vi "Deposit Funds.vi"(8 "error in":errorcluster, 9 "Amount":dbl, 10 "Account Number":string, 11 "Accounts File Path":path) -> (0 "error out":errorcluster, 3 "Account":T1)   [LabVIEW 2026]
doc: "Deposits Amount into an account. The CURRENT balance is read from the accounts file (Get Account.vi), Amount is added and the new balance is written back with Update Account Balance.vi; Account returns the updated record. An account number that is not in the file returns error 5003 and nothing is written. When error in carries an error the file is neither read nor written."
uses:
  Controls/ATM Account.ctl
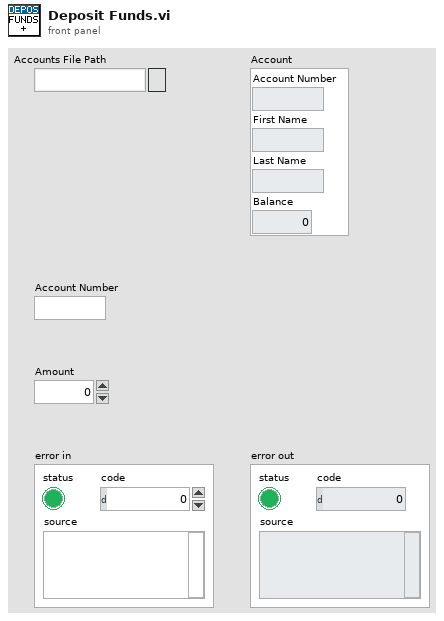
[diagram p1: front panel]
types:
  T1 = typedef "ATM Account.ctl" = cluster{"Account Number":string, "First Name":string, "Last Name":string, "Balance":dbl}
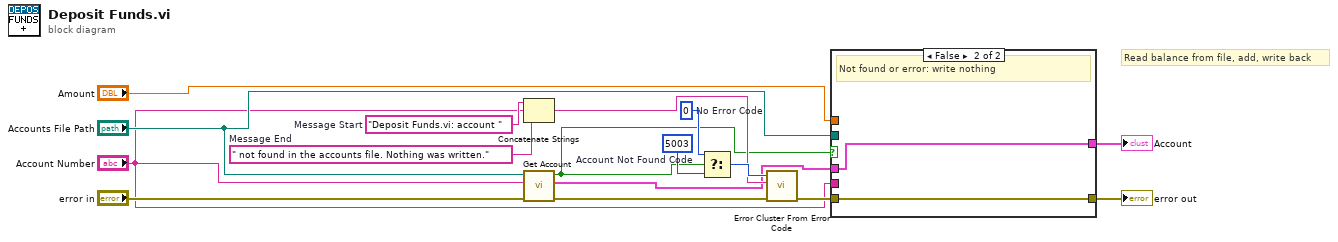
[diagram p0: block diagram]
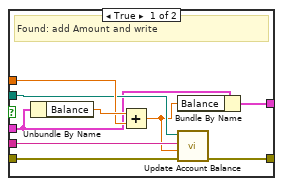
[diagram p2: hidden frame]
diagram:
  w12 = " not found in the accounts file. Nothing was written."  # Message End
  w13 = "Deposit Funds.vi: account "  # Message Start
  w14 = 5003  # Account Not Found Code
  w15 = 0  # No Error Code
  # "Read balance from file, add, write back"
  n1 = Concatenate Strings(w13, "Account Number", w12) -> (w10:string)
  n2 = call "Get Account.vi"("error in"="error in", "Account Number"="Account Number", "Accounts File Path"="Accounts File Path") -> ("error out"=w9:errorcluster, "Account"=w8:T1, "Account Found?"=w3:bool)  [unwired: 6 in]
  n3 = Select(t=w15, s=w3, f=w14) -> (s? t:f=w11:i32)
  n4 = call <vilib>:"Error Cluster From Error Code.vi"("error in (no error)"=w9, "error message (\"\")"=w10, "error code (0)"=w11) -> ("error out"=w7:errorcluster)  [unwired: 6 in]
  n5 = case shown="False" w3 {
    tunnel: w8 -> [w19 w27]
    tunnel: w7 -> [w21 w26]
    tunnel: "Accounts File Path" -> [w23 _]
    tunnel: "Account Number" -> [w22 _]
    tunnel: "Amount" -> [w24 _]
    tunnel: [w18 w27] -> w2
    tunnel: [w17 w26] -> w1
    frame True {
      # "Found: add Amount and write"
      n6 = Unbundle By Name(w19) -> ("Balance"=w25:dbl)
      n7 = Add(x=w25, y=w24) -> (x+y=w20:dbl)
      n8 = Bundle By Name(cluster=w19, "Balance"=w20) -> (w18:T1)
      n9 = call "Update Account Balance.vi"("error in"=w21, "New Balance"=w20, "Account Number"=w22, "Accounts File Path"=w23) -> ("error out"=w17:errorcluster)  [unwired: 7 in]
    }
    frame False {
      # "Not found or error: write nothing"
    }
  }
  "Account" <- w2
  "error out" <- w1
